vi "TCP Server Example.vi"() -> ()   [LabVIEW 2020]
uses:
  _Data Structures/TCP Server Public Connections Info Cluster.ctl
  JKI TCP Server.lvclass
panel:
  in  "Disconnect all clients?":bool
  out "Time Running (s)":dbl format="%#.0g"
  in  "max connections (0: no limit)":u32=2
  in  "stop":bool
  out "No. of Connections":u32
  out "Connections Info":T1[](array[typedef])
  in  "port":u16=50007
  # "Server Status"
  # "Server Config"
  # "-= INSTRUCTIONS =-\n\nOpen a command prompt and type:\n\nC:\\> telnet localhost 8080\n\nType: \"quit\", \"exit\", or \"bye\" to exit.\n\nTry connecting with multiple clients simultaneously.  Note that only one client is allowed to connect if the \"Connection Handler VI is not reentrant\".  Otherwise you are only limited by \"max connections\"."
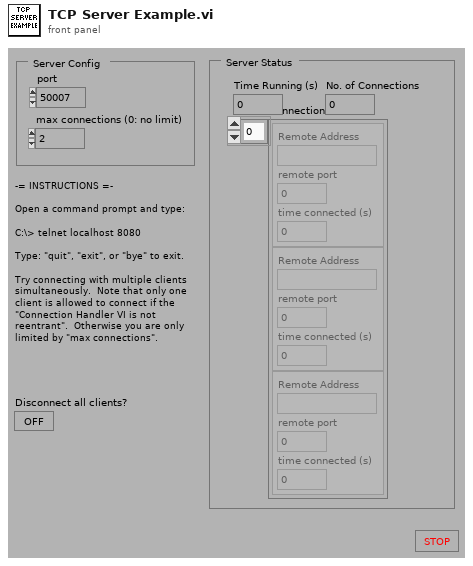
[diagram p1: front panel]
types:
  T1 = typedef "JKI TCP Server.lvclass/TCP Server Public Connections Info Cluster.ctl" = cluster{"Remote Address":string, "remote port":u16, "time connected (s)":dbl}
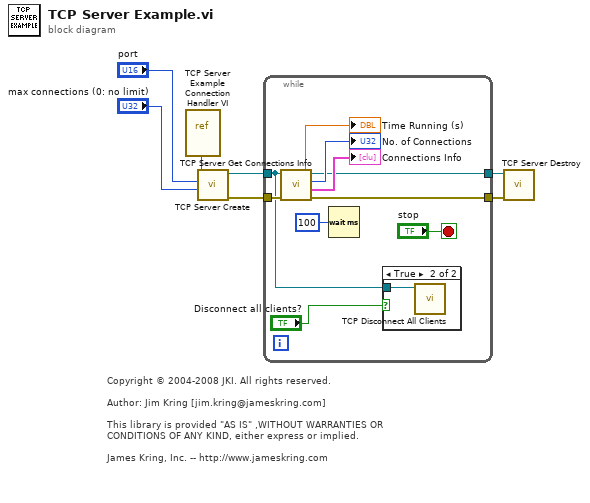
[diagram p0: block diagram]
diagram:
  # "Copyright © 2004-2008 JKI. All rights reserved.\n\nAuthor: Jim Kring [jim.kring@jameskring.com]\n\nThis library is provided \"AS IS\" ,WITHOUT WARRANTIES OR \nCONDITIONS OF ANY KIND, either express or implied.\n\nJames Kring, Inc. -- http://www.jameskring.com"
  n1 = vi-ref "TCP Server Example Connection Handler VI.vi"() -> ("vi reference"=w1:refnum<vi>)
  n2 = call "TCP Server Create.vi"("max connections (0: no limit)"="max connections (0: no limit)", "port"="port", "Connection Handler Call-Back VI RefNum"=w1) -> ("error out"=w6:errorcluster, "TCP Server RefNum"=w5:refnum<class "JKI TCP Server.lvclass">)  [unwired: 7 in]
  n3 = while {
    tunnel: w6 -> [w12]
    tunnel: w5 -> [w9]
    tunnel: [w11] -> w4
    tunnel: [w10] -> w3
    stop <- "stop" stop-if-true
    n4 = call "TCP Server Get Connections Info.vi"("error in (no error)"=w12, "TCP Server"=w9) -> ("error out"=w10:errorcluster, "Connections Info"=→"Connections Info":T1[], "Number of Connections"=→"No. of Connections":u32, "TCP Server out"=w11:refnum<class "JKI TCP Server.lvclass">, "time running (s)"=→"Time Running (s)":dbl)  [unwired: 5 in]
    n5 = Wait (ms)(milliseconds to wait=u32 100) -> ()  [unwired: 1 out]
    n6 = case shown="True" "Disconnect all clients?" {
      tunnel: w9 -> [_ w18]
      frame False {
      }
      frame True {
        n7 = call "TCP Disconnect All Clients.vi"("TCP Server"=w18) -> ()  [unwired: 9 in, 2 out]
      }
    }
  }
  n8 = call "TCP Server Destroy.vi"("error in (no error)"=w3, "TCP Server"=w4) -> ()  [unwired: 9 in, 1 out]
